vi "Func - LV runtime error handler_.vi"(7 "InstanceRef":T1, 8 "error in":bool, 10 "Gen CE error?":bool, 11 "LabVIEW error code":i32) -> (0 "error out":bool)   [LabVIEW 2021]
doc: "This VI handles errors returned by LabVIEW VIs and functions. Refer to the VI help for more details.\n\n::: CalcExpress Toolkit :::\nCopyright (c) 2000-2026 Konstantin Shifershteyn. All rights reserved."
uses:
  cetypes.llb/CalcExpress Instance RefNum.ctl
  <vilib>/Utility/error.llb/DialogType.ctl
  Func Globals xxx.vi
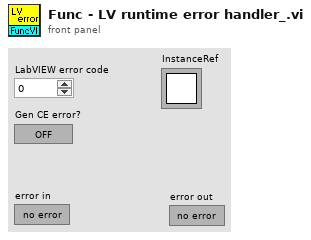
[diagram p1: front panel]
types:
  T1 = typedef "CalcExpress Instance RefNum.ctl" = refnum<k1>
  T2 = typedef "DialogType.ctl" = u16
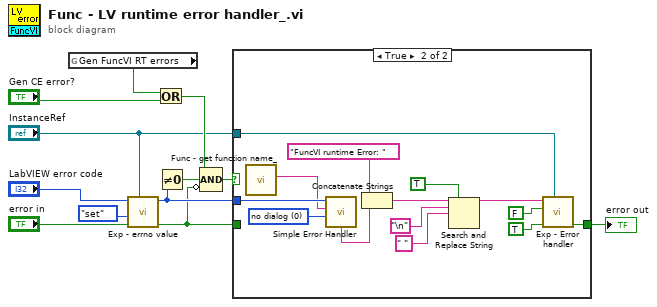
[diagram p0: block diagram]
diagram:
  n1 = global read "Func Globals xxx.vi" "Gen FuncVI RT errors"() -> (w1:bool)
  n2 = call "Exp - errno value.vi"("InstanceRef"="InstanceRef", "error in"="error in", "action"=enum32{"get", "set"}."set", "errno value"="LabVIEW error code") -> ("error out"=w3:bool, "errno value out"=w9:i32)  [unwired: 3 in, 1 out]
  n3 = Or(x=w1, y="Gen CE error?") -> (x .or. y?=w12:bool)
  n4 = Not Equal To 0?(x=w9) -> (x != 0?=w5:bool)
  n5 = Compound Arithmetic op=AND(w12, w5, invert w3) -> (w11:bool)
  n6 = case shown="True" w11 {
    tunnel: w9 -> [_ w27]
    tunnel: [w13 w26] -> w8
    tunnel: w3 -> [w13 _]
    tunnel: "InstanceRef" -> [_ w20]
    frame False {
    }
    frame True {
      w14 = T2 0 items=["no dialog", "OK message", "continue or stop message", "OK message + warnings", "continue/stop + warnings"] ("type of dialog (OK msg:1)")
      n7 = call "Func - get function name_.vi"() -> ("FuncVI name"=w22:string)  [unwired: 9 in, 2 out]
      n8 = call <vilib>:"Simple Error Handler.vi"("error code (no error:0)"=w27, "error source (\" \")"=w22, "type of dialog (OK msg:1)"=w14) -> ("message"=w24:string)  [unwired: 2 in, 4 out]
      n9 = Concatenate Strings("FuncVI runtime Error: ", w24) -> (w19:string)
      n10 = Search and Replace String(replace all?=TRUE, input string=w19, search string="\n", replace string=" " ("replace string (\"\")")) -> (result string=w15:string)  [unwired: 4 in, 3 out]
      n11 = call "Exp - Error handler.vi"("InstanceRef"=w20, "error in"=TRUE, "add FuncName (T)"=FALSE, "error message in"=w15) -> ("error out"=w26:bool)  [unwired: 5 in, 2 out]
    }
  }
  "error out" <- w8
